vi "Name Value Remove Group.vi"(0 "Tags Array":string[][][](array[string]), 7 "Boolean Refs Array":refnum<vi>[](array[refnum]), 11 "Group Index":i32) -> (4 "Updated Tag Array":string[][][](array[string]), 8 "Update Index":i32, 15 "Current Tags":string[][](array[string]))   [LabVIEW 2020]
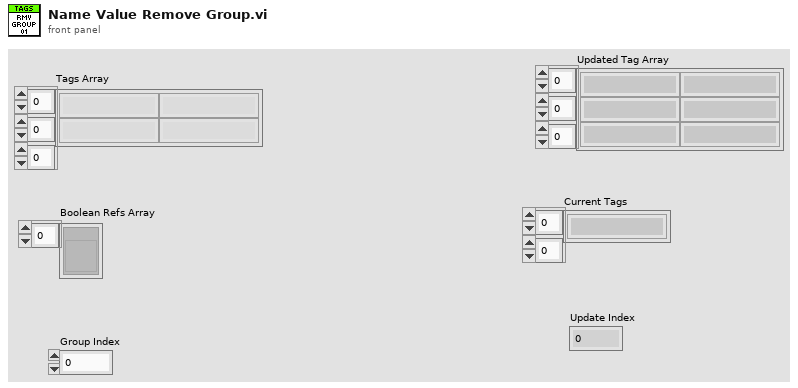
[diagram p1: front panel]
types:
  T1 = enum8{"Enabled", "Disabled", "Disabled and Grayed Out"}
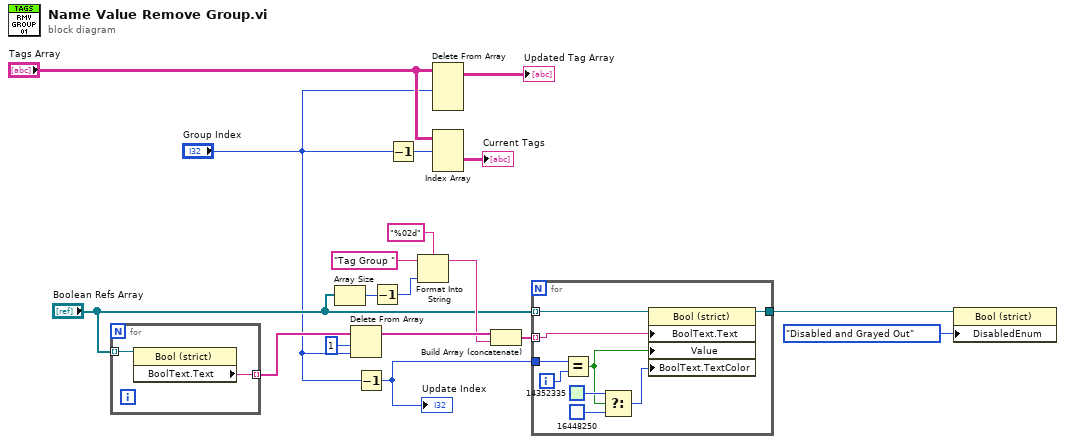
[diagram p0: block diagram]
diagram:
  n1 = for {
    tunnel: "Boolean Refs Array" -> [w20] mode=indexing
    tunnel: [w19] -> w4 mode=indexing
    n2 = property class="Bool (strict)"(reference=w20) -> ("BoolText.Text"=w19:string)  [unwired: 1 in, 2 out]
  }
  n3 = Array Size(array="Boolean Refs Array") -> (size(s)=w14:i32)
  n4 = Delete From Array(array=w4, length=1, index="Group Index") -> (array with subset deleted=w17:string[])  [unwired: 1 out]
  n5 = Decrement(x="Group Index") -> (x-1=w8:i32)
  "Update Index" <- w8
  n6 = Decrement(x=w14) -> (x-1=w11:i32)
  n7 = Decrement(x="Group Index") -> (x-1=w2:i32)
  n8 = Format Into String(format string="%02d", initial string="Tag Group ", w11) -> (resulting string=w13:string)  [unwired: 1 in, 1 out]
  n9 = Delete From Array(array="Tags Array", index (dim 0)="Group Index") -> (array with subset deleted=→"Updated Tag Array":string[][][])  [unwired: 3 in, 1 out]
  n10 = Index Array(array="Tags Array", index (dim 0)=w2) -> (element=→"Current Tags":string[][])  [unwired: 2 in]
  n11 = Build Array (concatenate)(w17, w13) -> (w12:string[])
  n12 = for {
    tunnel: "Boolean Refs Array" -> [w29] mode=indexing
    tunnel: w12 -> [w26] mode=indexing
    tunnel: w8 -> [w28]
    tunnel: [w21] -> w9
    i -> [w27]
    n13 = Equal?(x=w28, y=w27) -> (x = y?=w23:bool)
    n14 = Select(t=u32 14352335 ("Color Box"), s=w23, f=u32 16448250) -> (s? t:f=w22:u32)
    n15 = property class="Bool (strict)"(reference=w29, "BoolText.Text"=w26, "Value"=w23, "BoolText.TextColor"=w22) -> (reference out=w21:refnum<vi>)  [unwired: 1 in, 1 out]
  }
  n16 = property class="Bool (strict)"(reference=w9, "DisabledEnum"=T1."Disabled and Grayed Out" ("Disabled")) -> ()  [unwired: 1 in, 2 out]
